vi "rose.vi"() -> ()   [LabVIEW 2021]
uses:
  <vilib>/Utility/miscctls.llb/LV3DPointTypeDef.ctl
  <vilib>/Utility/miscctls.llb/LVRGBAColorTypeDef.ctl
  <vilib>/picture/3D Picture Control/Object/Create Object (name).vi
  <vilib>/picture/3D Picture Control/Helpers/Apply Texture (no reference).vi
  <vilib>/picture/3D Picture Control/Helpers/Set Light (no reference).vi
  <vilib>/picture/3D Picture Control/NI_3D Picture Control.lvlib
panel:
  in  "stop":bool
  out "3D Picture":refnum<vi>(3d-picture)
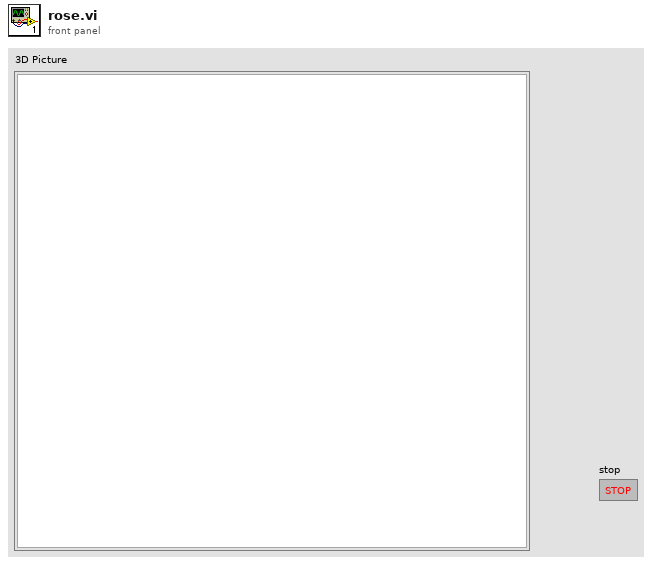
[diagram p1: front panel]
types:
  T1 = enum16{"Normal Bin", "Opaque Bin", "Transparent Bin"}
  T2 = enum16{"Inherit Value", "No Culling", "Cull Back Face", "Cull Front Face", "Cull Both Faces"}
  T3 = enum16{"Inherit Value", "Points", "Wireframe", "Polygons"}
  T4 = typedef "LVRGBAColorTypeDef.ctl" = cluster{"Red":sgl, "Green":sgl, "Blue":sgl, "Alpha":sgl}
  T5 = enum16{"Inherit Material", "Use entire Material", "Ignore Ambient", "Ignore Diffuse", "Ignore Specular", "Ignore Emission", "Ignore Ambient and Diffuse"}
  T6 = typedef "LV3DPointTypeDef.ctl" = cluster{"X":sgl, "Y":sgl, "Z":sgl}
  T7 = enum16{"As a Decal", "With Modulation", "With Blending", "As a replacement"}
  T8 = typedef "imagedata.ctl" = cluster{"image type":i32, "image depth":i32, "image":u8[], "mask":u8[], "colors":u32[], "Rectangle":cluster{"left":i16, "top":i16, "right":i16, "bottom":i16}}
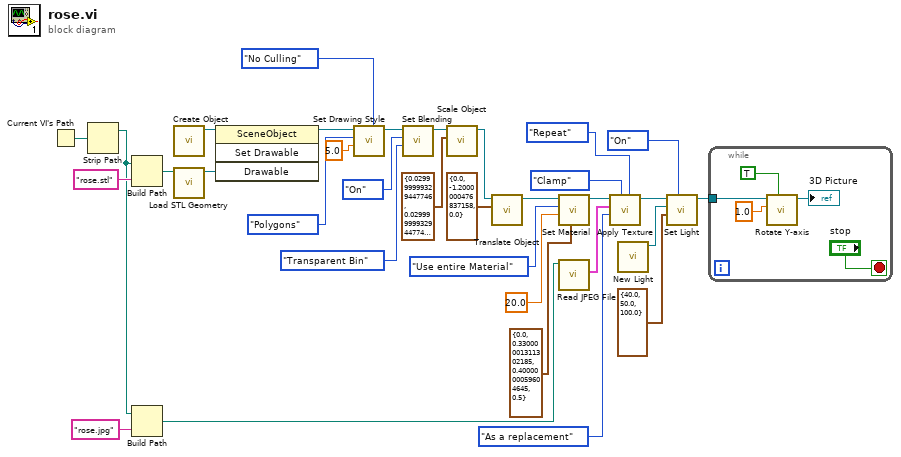
[diagram p0: block diagram]
diagram:
  n1 = Current VI's Path() -> (path=w32:path)
  n2 = Strip Path(path=w32) -> (stripped path=w24:path)  [unwired: 1 out]
  n3 = Build Path(base path=w24, name or relative path="rose.stl") -> (appended path=w31:path)
  n4 = Build Path(base path=w24, name or relative path="rose.jpg") -> (appended path=w23:path)
  n5 = call-poly <vilib>:"Create Object.vi"() -> ("Scene:New Object"=w30:refnum<vi>)  [unwired: 10 in, 1 out]
  n6 = call <vilib>:"Load STL Geometry.vi"("Model File"=w31) -> ("New Mesh Refnum"=w28:refnum<vi>)  [unwired: 9 in, 1 out]
  n7 = invoke class="SceneObject" method="Set Drawable"(reference=w30, "Drawable"=w28) -> (reference out=w8:refnum<vi>)  [unwired: 2 in, 3 out]
  n8 = call <vilib>:"Set Drawing Style.vi"("Face Culling Mode"=T2."No Culling", "Size"=5.0, "Mode"=T3."Polygons", "Scene Object In"=w8) -> ("Scene Object Out"=w4:refnum<vi>)  [unwired: 6 in, 1 out]
  n9 = call <vilib>:"Set Blending.vi"("Bin"=T1."Transparent Bin", "Mode"=enum16{"Inherit Value", "Off", "On"}."On", "Scene Object In"=w4) -> ("Scene Object Out"=w3:refnum<vi>)  [unwired: 7 in, 1 out]
  n10 = call <vilib>:"Scale Object.vi"("Scale"=cluster{"X":sgl, "Y":sgl, "Z":sgl} {"X"=0.03, "Y"=0.03, "Z"=0.03}, "Scene.Object In"=w3) -> ("Scene.Object Out"=w27:refnum<vi>)  [unwired: 8 in, 1 out]
  n11 = call <vilib>:"Translate Object.vi"("Translation"=cluster{"X":sgl, "Y":sgl, "Z":sgl} {"X"=0.0, "Y"=-1.2, "Z"=0.0}, "Scene.Object In"=w27) -> ("Scene.Object Out"=w13:refnum<vi>)  [unwired: 8 in, 1 out]
  n12 = call <vilib>:"Set Material.vi"("Emission"=T4 {"Red"=0.0, "Green"=0.33, "Blue"=0.4, "Alpha"=0.5}, "Shininess"=sgl 20.0, "Color Mode"=T5."Use entire Material", "Scene Object In"=w13) -> ("Scene Object Out"=w10:refnum<vi>)  [unwired: 6 in, 1 out]
  n13 = call <vilib>:"Read JPEG File.vi"("path to JPEG file"=w23) -> ("image data"=w22:T8)  [unwired: 8 in, 2 out]
  n14 = call-poly <vilib>:"Apply Texture.vi"("Vertical Wrap Mode"=enum16{"Clamp", "Repeat"}."Repeat", "Horizontal Wrap Mode"=enum16{"Clamp", "Repeat"}."Clamp", "Apply Mode"=T7."As a replacement", "Image Data"=w22, "Scene Object In"=w10) -> ("Scene Object Out"=w18:refnum<vi>)  [unwired: 5 in, 1 out]
  n15 = call <vilib>:"New Light.vi"() -> ("New Light Refnum"=w17:refnum<vi>)  [unwired: 10 in, 1 out]
  n16 = call-poly <vilib>:"Set Light.vi"("Light State"=enum16{"Inherit Value", "Off", "On"}."On", "Position"=T6 {"X"=40.0, "Y"=50.0, "Z"=100.0}, "Light Refnum In"=w17, "Scene Object In"=w18) -> ("Scene Object Out"=w15:refnum<vi>)  [unwired: 6 in, 1 out]
  n17 = while {
    tunnel: w15 -> [w38]
    stop <- "stop" stop-if-true
    n18 = call <vilib>:"Rotate Y-axis.vi"("Relative?"=TRUE, "angle"=1.0, "Scene Object In"=w38) -> ("Scene Object Out"=→"3D Picture":refnum<vi>)  [unwired: 7 in, 1 out]
  }
